vi "virtuino_labview.vi"() -> ()   [LabVIEW 2025]
panel:
  out "led":bool
  out "Thermometer":dbl(slide) scale=0.0..100.0
  out "data out":string
  in  "remote port or service name":u16
  in  "address":string
  in  "stop":bool
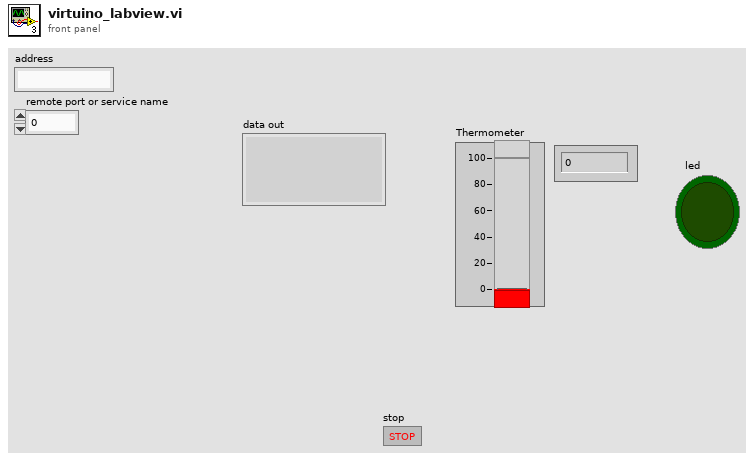
[diagram p1: front panel]
types:
  T1 = enum16{"Standard", "Buffered", "CRLF", "Immediate"}
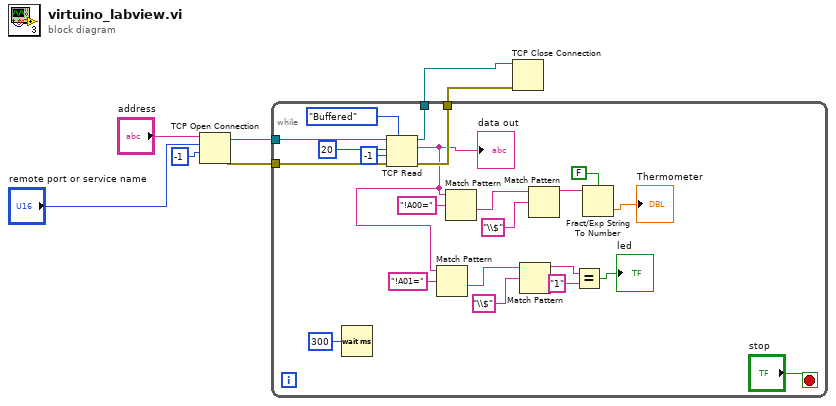
[diagram p0: block diagram]
diagram:
  n1 = TCP Open Connection(address="address", remote port or service name="remote port or service name", timeout ms (60000)=-1) -> (connection ID=w4:refnum<k5>, error out=w3:errorcluster)  [unwired: 2 in]
  n2 = while {
    tunnel: w4 -> [w28]
    tunnel: w3 -> [w27]
    tunnel: [w23] -> w2
    tunnel: [w22] -> w1
    stop <- "stop" stop-if-true
    n3 = Wait (ms)(milliseconds to wait=u32 300) -> ()  [unwired: 1 out]
    n4 = TCP Read(connection ID=w28, bytes to read=20, error in (no error)=w27, 7:T1."Buffered" ("mode (standard)"), 9:-1 ("timeout ms (25000)")) -> (connection ID out=w22:refnum<k5>, data out=w11:string, error out=w23:errorcluster)
    "data out" <- w11
    n5 = Match Pattern(string=w11, regular expression="!A01=") -> (after substring=w13:string)  [unwired: 1 in, 3 out]
    n6 = Match Pattern(string=w11, regular expression="!A00=") -> (after substring=w19:string)  [unwired: 1 in, 3 out]
    n7 = Match Pattern(string=w13, regular expression="\\$") -> (before substring=w10:string)  [unwired: 1 in, 3 out]
    n8 = Match Pattern(string=w19, regular expression="\\$") -> (before substring=w17:string)  [unwired: 1 in, 3 out]
    n9 = Equal?(x=w10, y="1") -> (x = y?=→"led":bool)
    n10 = Fract/Exp String To Number(use system decimal point (T)=FALSE, string=w17) -> (number=→"Thermometer":dbl)  [unwired: 2 in, 1 out]
  }
  n11 = TCP Close Connection(connection ID=w1, error in (no error)=w2) -> ()  [unwired: 1 in, 2 out]
